vi "LabVIEW.Service.Create a local report file.vi"(7 "Folder path":path, 8 "Fehler (Eingang)":errorcluster, 10 "Server type":string="SNDB_Se", 11 "Failed report text":string) -> (0 "error out":errorcluster caption="Fehler (Ausgang)", 3 "Successful?":bool, 5 "Path":string)   [LabVIEW 2026]
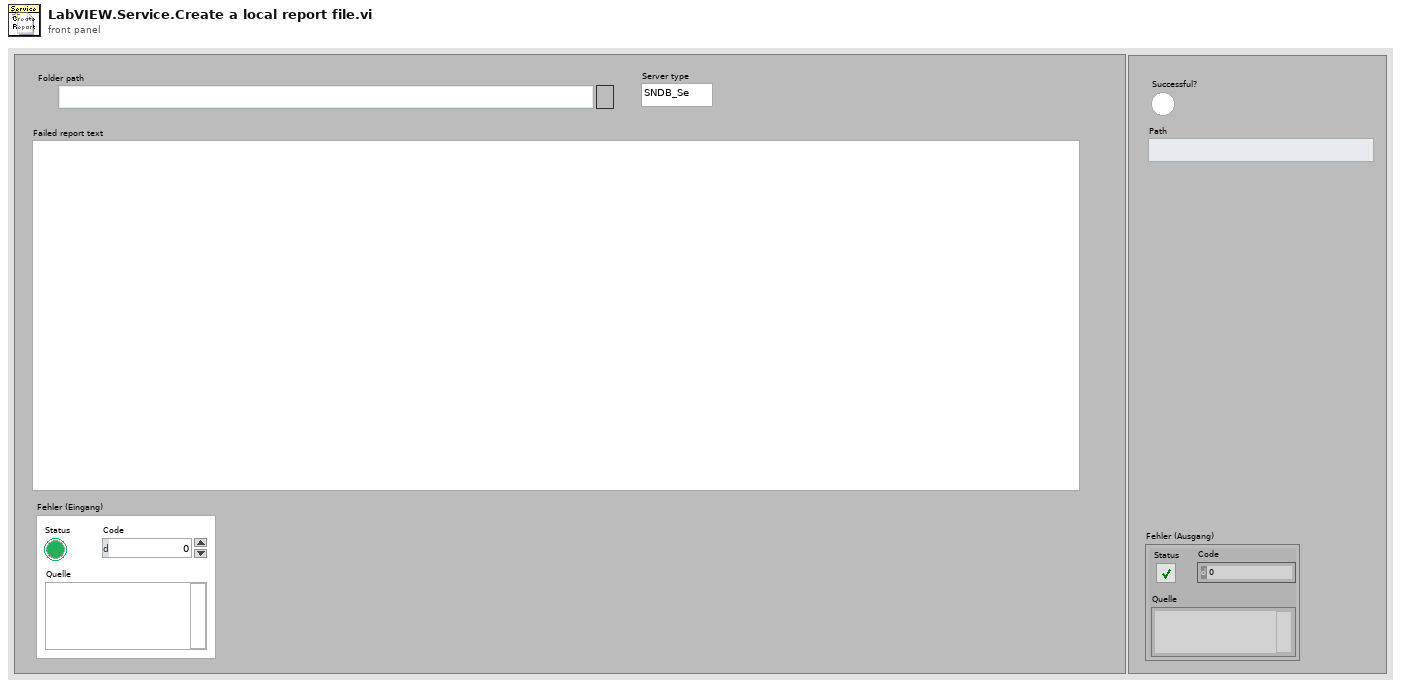
[diagram p1: front panel]
types:
  T1 = enum16{"open", "replace", "create", "open or create", "replace or create", "replace or create with confirmation"}
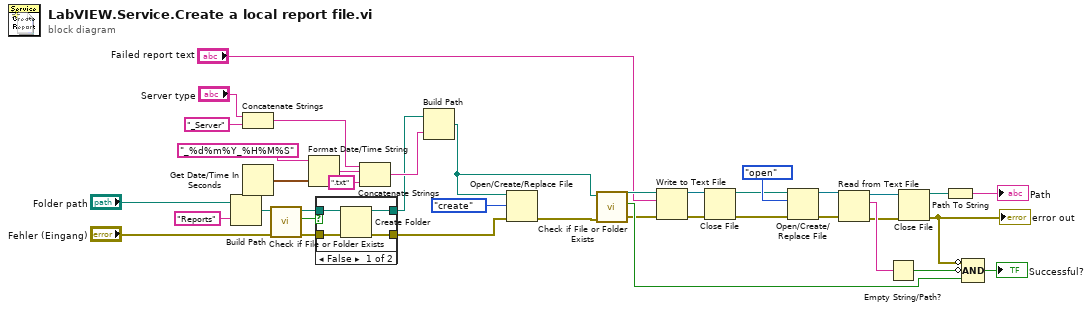
[diagram p0: block diagram]
diagram:
  n1 = Build Path(base path="Folder path", name or relative path="Reports") -> (appended path=w8:path)
  n2 = Concatenate Strings("Server type", "_Server" ("String")) -> (w10:string)
  n3 = Get Date/Time In Seconds() -> (seconds since 1Jan1904=w38:timestamp)
  n4 = call <vilib>:"Check if File or Folder Exists.vi"("error in (no error)"="Fehler (Eingang)", "path"=w8) -> ("error out"=w9:errorcluster, "file or folder exists?"=w6:bool, "dup path"=w7:path)  [unwired: 7 in]
  n5 = Format Date/Time String(time format string (%c)="_%d%m%Y_%H%M%S" ("Zeitformatierungs-String (%c)"), seconds (now)=w38) -> (date/time string=w37:string)  [unwired: 1 in]
  n6 = case shown="False" w6 {
    tunnel: w7 -> [w43 w45]
    tunnel: [w42 w44] -> w2
    tunnel: [w41 w45] -> w1
    tunnel: w9 -> [w40 w44]
    frame False {
      n7 = Create Folder(path (use dialog)=w43, error in=w40) -> (created path=w41:path, error out=w42:errorcluster)  [unwired: 1 in, 1 out]
    }
    frame True {
    }
  }
  n8 = Concatenate Strings(w10, w37, ".txt" ("String")) -> (w35:string)
  n9 = Build Path(base path=w1, name or relative path=w35) -> (appended path=w20:path)
  n10 = Open/Create/Replace File(file path (use dialog)=w20, error in=w2, operation (0:open)=T1."create" ("Operation (0:open)")) -> (error out=w21:errorcluster)  [unwired: 3 in, 2 out]
  n11 = call <vilib>:"Check if File or Folder Exists.vi"("error in (no error)"=w21, "path"=w20) -> ("error out"=w25:errorcluster, "file or folder exists?"=w28:bool, "dup path"=w26:path)  [unwired: 7 in]
  n12 = Write to Text File(file (use dialog)=w26, text="Failed report text", error in=w25) -> (refnum out=w18:refnum<file>, error out=w19:errorcluster)  [unwired: 1 in, 1 out]
  n13 = Close File(refnum=w18, error in=w19) -> (path=w16:path, error out=w15:errorcluster)
  n14 = Open/Create/Replace File(file path (use dialog)=w16, error in=w15, operation (0:open)=T1."open" ("Operation (0:open)")) -> (refnum out=w14:refnum<file>, error out=w13:errorcluster)  [unwired: 3 in, 1 out]
  n15 = Read from Text File(file (use dialog)=w14, error in=w13) -> (refnum out=w32:refnum<file>, text=w33:string, error out=w31:errorcluster)  [unwired: 2 in, 1 out]
  n16 = Empty String/Path?(string/path=w33) -> (empty?=w29:bool)
  n17 = Close File(refnum=w32, error in=w31) -> (path=w23:path, error out=w30:errorcluster)
  "error out" <- w30
  n18 = Path To String(path=w23) -> (string=→"Path":string)
  n19 = Compound Arithmetic op=AND ("Mehrfacharithmetik")(invert w30, invert w29, w28) -> (→"Successful?":bool)
